vi "Input Required Response.vi"(8 "_meta":string, 9 "input requests":string, 10 "id":string, 11 "method":string) -> (2 "input required?":bool, 3 "response":string)   [LabVIEW 2020, in "MCP Server.lvlib"]
doc: "Builds the answer to a modern tools/call for which the tool registered questions (Ask User.vi): {\"jsonrpc\":\"2.0\",\"id\":<id>,\"result\":{\"resultType\":\"input_required\",\"inputRequests\":<input requests>,\"_meta\":<_meta>}}. input required? is TRUE when method is tools/call and input requests is not empty. Used by Complete Modern MCP Result.vi."
uses:
  MCP Server.lvlib
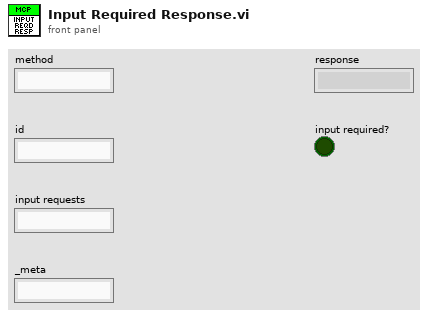
[diagram p1: front panel]
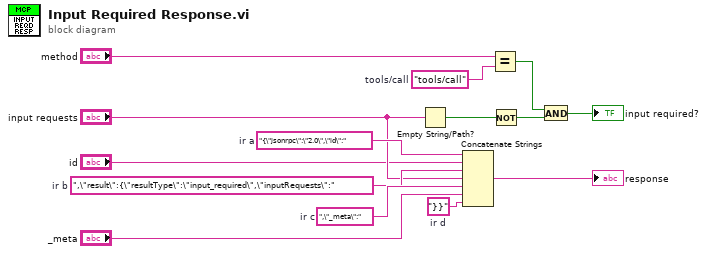
[diagram p0: block diagram]
diagram:
  w9 = "}}"  # ir d
  w8 = ",\"_meta\":"  # ir c
  w7 = ",\"result\":{\"resultType\":\"input_required\",\"inputRequests\":"  # ir b
  w6 = "{\"jsonrpc\":\"2.0\",\"id\":"  # ir a
  w5 = "tools/call"  # tools/call
  n1 = Empty String/Path?(string/path="input requests") -> (empty?=w11:bool)
  n2 = Concatenate Strings(w6, "id", w7, "input requests", w8, "_meta", w9) -> (→"response":string)
  n3 = Equal?(x="method", y=w5) -> (x = y?=w10:bool)
  n4 = Not(x=w11) -> (.not. x?=w12:bool)
  n5 = And(x=w10, y=w12) -> (x .and. y?=→"input required?":bool)
